vi "c Spark Get Periodic Status1.vi"(8 "error in (no error)":errorcluster, 10 "spart_status_1":T1, 11 "handle":T2) -> (0 "error out":errorcluster, 1 "function return":T3, 2 "spart_status_1":T1, 3 "handle out":T2)   [LabVIEW 2023, in "REVLibDriver.lvlib"]
doc: "c_REVLib_ErrorCode c_Spark_GetPeriodicStatus1(\n c_Spark_handle handle, c_Spark_PeriodicStatus1* rawframe);"
uses:
  <vilib>/REVLibDriver/REVLibDriver.lvlib
  <vilib>/REVLibDriver/subvi/RevLibError.ctl
  <vilib>/REV Custom Controls/c_Spark_handle.ctl
  <vilib>/REV Custom Controls/c_Spark_PeriodicStatus1.ctl
  REVLibDriver.so
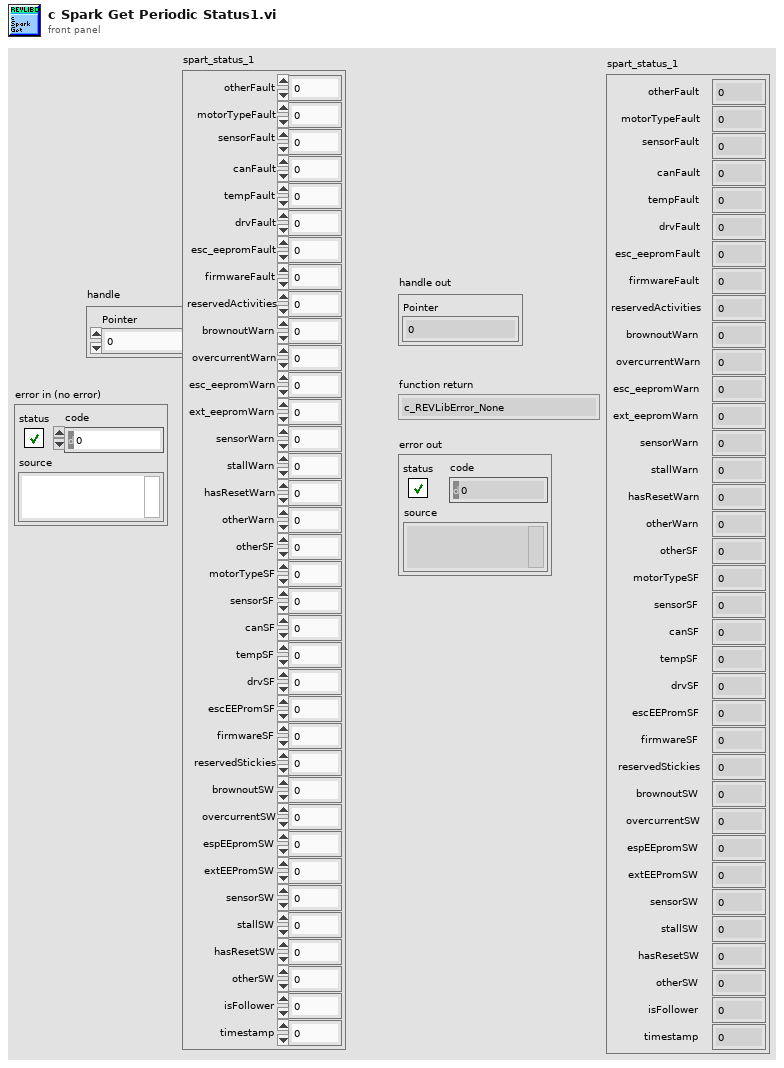
[diagram p1: front panel]
types:
  T1 = typedef "REVLibDriver.lvlib/c_Spark_PeriodicStatus1.ctl" = cluster{"otherFault":u8, "motorTypeFault":u8, "sensorFault":u8, "canFault":u8, "tempFault":u8, "drvFault":u8, "esc_eepromFault":u8, "firmwareFault":u8, "reservedActivities":u8, "brownoutWarn":u8, "overcurrentWarn":u8, "esc_eepromWarn":u8, "ext_eepromWarn":u8, "sensorWarn":u8, "stallWarn":u8, "hasResetWarn":u8, "otherWarn":u8, "otherSF":u8, "motorTypeSF":u8, "sensorSF":u8, "canSF":u8, "tempSF":u8, "drvSF":u8, "escEEPromSF":u8, "firmwareSF":u8, "reservedStickies":u8, "brownoutSW":u8, "overcurrentSW":u8, "espEEpromSW":u8, "extEEPromSW":u8, "sensorSW":u8, "stallSW":u8, "hasResetSW":u8, "otherSW":u8, "isFollower":u8, "timestamp":u64}
  T2 = typedef "REVLibDriver.lvlib/c_Spark_handle.ctl" = cluster{"Pointer":u64}
  T3 = typedef "REVLibDriver.lvlib/RevLibError.ctl" = enum16{"c_REVLibError_None", "c_REVLibError_General", "c_REVLibError_CANTimeout", "c_REVLibError_NotImplemented", "c_REVLibError_HAL", "c_REVLibError_CantFindFirmware", "c_REVLibError_FirmwareTooOld", "c_REVLibError_FirmwareTooNew", "c_REVLibError_ParamInvalidID", "c_REVLibError_ParamMismatchType", "c_REVLibError_ParamAccessMode", "c_REVLibError_ParamInvalid", "c_REVLibError_ParamNotImplementedDeprecated", "c_REVLibError_FollowConfigMismatch", "c_REVLibError_Invalid", "c_REVLibError_SetpointOutOfRange", "c_REVLibError_Unknown", "c_REVLibError_CANDisconnected", "c_REVLibError_DuplicateCANId", "c_REVLibError_InvalidCANId", "c_REVLibError_SparkMaxDataPortAlreadyConfiguredDifferently", "c_REVLibError_SparkFlexBrushedWithoutDock", "c_REVLibError_InvalidBrushlessEncoderConfiguration", "c_REVLibError_FeedbackSensorIncompatibleWithDataPortConfig", "c_REVLibError_ParamInvalidChannel", "c_REVLibError_ParamInvalidValue", "c_REVLibError_CannotPersistParametersWhileEnabled", "c_REVLibError_NotReadyToReceiveCommand", "c_REVLibError_NumCodes"}
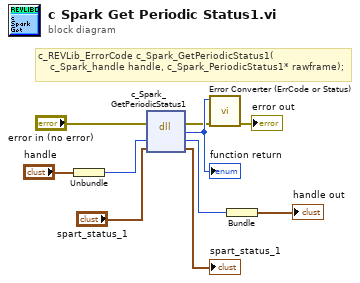
[diagram p0: block diagram]
diagram:
  # "c_REVLib_ErrorCode c_Spark_GetPeriodicStatus1(\n    c_Spark_handle handle, c_Spark_PeriodicStatus1* rawframe);"
  n1 = Unbundle("handle") -> ("Pointer"=w2:u64)
  n2 = dll-call lib="REVLibDriver.*" fn="c_Spark_GetPeriodicStatus1"(error in="error in (no error)", "handle"=w2, "rawframe"="spart_status_1") -> (error out=w4:errorcluster, "return type"=w10:u32, "handle"=w8:u64, "rawframe"=→"spart_status_1":T1)  [unwired: 2 in, 1 out]
  "function return" <- w10
  n3 = call <vilib>:"Error Converter (ErrCode or Status).vi"("error in (no error)"=w4, "error code"=w10) -> ("error out"=→"error out":errorcluster)  [unwired: 9 in]
  n4 = Bundle("handle"=w8) -> (→"handle out":cluster{"handle":u64})  [unwired: 1 in]
